vi "Queue Inspection.vi"(8 "error in (no error)":errorcluster, 11 "Priority Queue in":refnum<class "Message Priority Queue.lvclass">) -> (0 "error out":errorcluster, 1 "Element Names":string[](array[string]), 2 "# elements in queue":i32, 3 "Priority Queue out":refnum<class "Message Priority Queue.lvclass">)   [LabVIEW 2020, in "Actor Framework.lvlib" / "Message Priority Queue.lvclass"]
uses:
  Message Priority Queue.lvclass
  Message Priority Queue.lvclass/Message Priority Queue.ctl
  Message/Message.lvclass
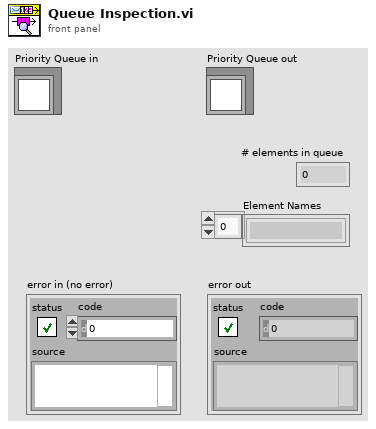
[diagram p1: front panel]
types:
  T1 = typedef "Actor Framework.lvlib/Message Priority Queue.lvclass/DVR Contents.ctl" = cluster{"# Waiting":u32, "Buffers":refnum<queue>[], "Wait Msg":refnum<queue>, "Wait Prior":refnum<queue>}
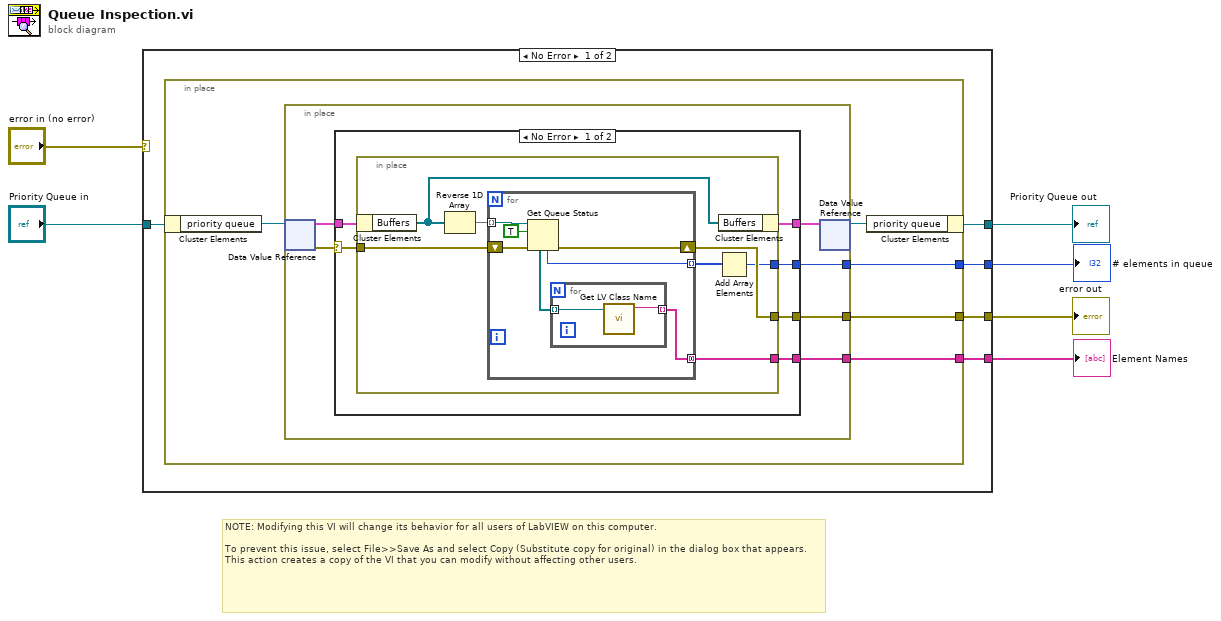
[diagram p0: block diagram]
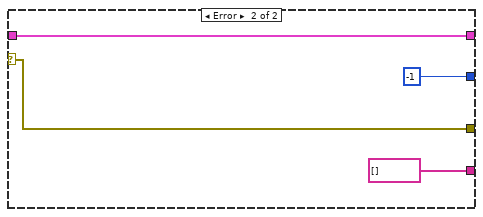
[diagram p2: hidden frame]
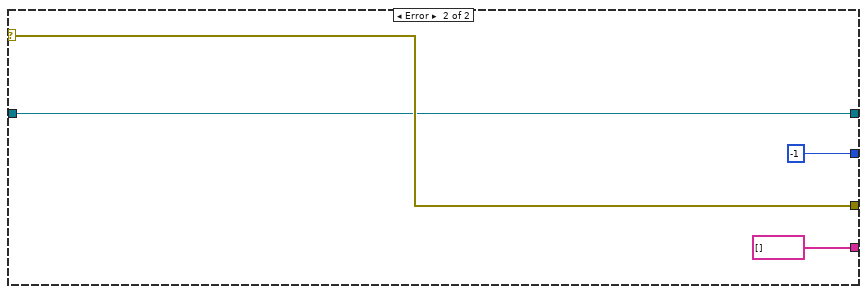
[diagram p3: hidden frame]
diagram:
  # "NOTE: Modifying this VI will change its behavior for all users of LabVIEW on this computer.\n\nTo prevent this issue, select File>>Save As and select Copy (Substitute copy for original) in the dialog box that appears. This action creates a copy of the VI that you can modify without affecting other users."
  n1 = case shown="No Error" "error in (no error)" {
    selector: "error in (no error)" -> [_ w52]
    tunnel: "Priority Queue in" -> [w11 w51]
    tunnel: [w10 w52] -> w4
    tunnel: [w9 w51] -> w3
    tunnel: [w8 -1 ("# elements in queue")] -> w2
    tunnel: [w7 string[] []] -> w1
    frame No Error {
      n2 = in-place {
        in-place-border: [w14] -> w10
        in-place-border: [w13] -> w8
        in-place-border: [w12] -> w7
        n3 = in-place-cluster #1(w11) -> ("priority queue"=w16:refnum<data-value>)
        n4 = in-place {
          in-place-border: [w19] -> w14
          in-place-border: [w18] -> w13
          in-place-border: [w17] -> w12
          n5 = in-place-dvr #2(w16) -> (w21:T1, w22:errorcluster)
          n6 = case shown="No Error" w22 {
            selector: w22 -> [w26 w47]
            tunnel: w21 -> [w28 w48]
            tunnel: [w27 w48] -> w20
            tunnel: [w25 w47] -> w19
            tunnel: [w24 -1 ("# elements in queue")] -> w18
            tunnel: [w23 string[] []] -> w17
            frame No Error {
              n7 = in-place {
                in-place-border: w26 -> [w34]
                in-place-border: [w33] -> w25
                in-place-border: [w30] -> w24
                in-place-border: [w29] -> w23
                n8 = in-place-cluster #3(w28) -> ("Buffers"=w35:refnum<queue>[])
                n9 = Reverse 1D Array(array=w35) -> (reversed array=w32:refnum<queue>[])
                n10 = for {
                  tunnel: w32 -> [w42] mode=indexing
                  shift-right: [w40] -> w33
                  shift-left: w34 -> [w41]
                  tunnel: [w39] -> w31 mode=indexing
                  tunnel: [w37] -> w29 mode=concatenating
                  n11 = Get Queue Status(queue=w42, return elements? (F)=TRUE, error in (no error)=w41) -> (error out=w40:errorcluster, # elements in queue=w39:i32, elements=w38:refnum<class "Message.lvclass">[])  [unwired: 5 out]
                  n12 = for {
                    tunnel: w38 -> [w44] mode=indexing
                    tunnel: [w43] -> w37 mode=indexing
                    n13 = call <vilib>:"Get LV Class Name.vi"("object"=w44) -> ("class name"=w43:string)  [unwired: 9 in, 1 out]
                  }
                }
                n14 = in-place-cluster #3("Buffers"=w35) -> (w27:T1)
                n15 = Add Array Elements(numeric array=w31) -> (sum=w30:i32)
              }
            }
            frame Error {
            }
          }
          n16 = in-place-dvr #2(w20) -> (w15:refnum<data-value>)  [unwired: 1 out]
        }
        n17 = in-place-cluster #1("priority queue"=w15) -> (w9:refnum<class "Message Priority Queue.lvclass">)
      }
    }
    frame Error {
    }
  }
  "Priority Queue out" <- w3
  "error out" <- w4
  "# elements in queue" <- w2
  "Element Names" <- w1
